vi "OwnCompat20261012_Native_GetEventInfo_v2.vi"() -> ()   [LabVIEW 2024]
panel:
  out "error out":errorcluster caption="错误输出"
  out "terminal_ids":u32[](array[numeric])
  in  "terminal_ids type":u32
  out "frame_ids":u32[](array[numeric])
  in  "frame_ids type":u32
  in  "event_id":u32
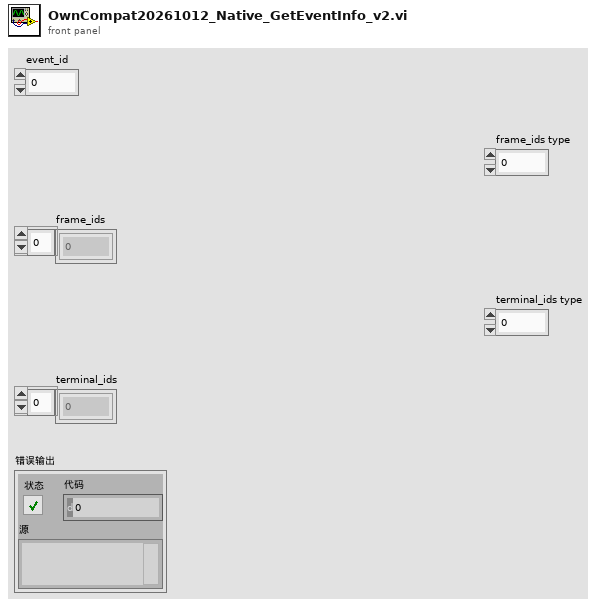
[diagram p1: front panel]
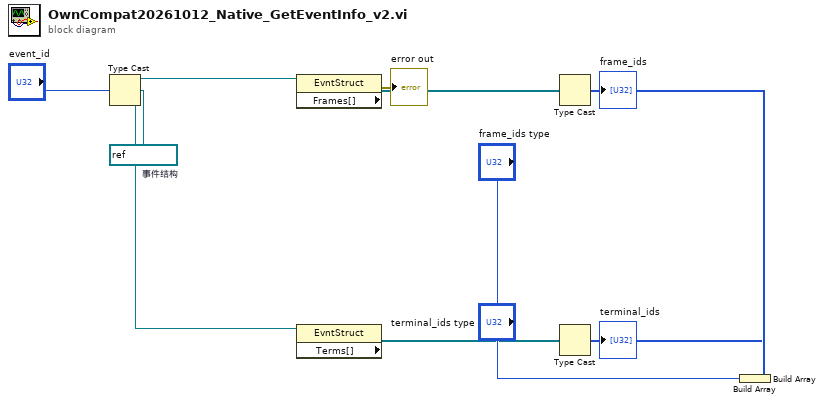
[diagram p0: block diagram]
diagram:
  w11 = refnum<vi> refnum  # 事件结构
  n1 = Type Cast ("强制类型转换")(type=w11, x="event_id") -> (*(type *) &x=w10:refnum<vi>)
  n2 = property on="属性节点" class="EvntStruct"(reference=w10) -> (error out=→"error out":errorcluster, "Frames[]"=w9:refnum<vi>[])  [unwired: 1 in, 1 out]
  n3 = property on="属性节点" class="EvntStruct"(reference=w10) -> ("Terms[]"=w5:refnum<vi>[])  [unwired: 1 in, 2 out]
  n4 = Build Array ("创建数组")("terminal_ids type") -> (w3:u32[])
  n5 = Type Cast ("强制类型转换")(type=w3, x=w5) -> (*(type *) &x=→"terminal_ids":u32[])
  n6 = Build Array ("创建数组")("frame_ids type") -> (w7:u32[])
  n7 = Type Cast ("强制类型转换")(type=w7, x=w9) -> (*(type *) &x=→"frame_ids":u32[])
